vi "GT_Monitor.vi"() -> ()   [LabVIEW 2026]
doc: "Use this template to build a VI to use as a subVI."
panel:
  out "error out":errorcluster
  in  "stop":bool
  out "Right Step Text":string
  out "Status":T1
  in  "PLC Port":string
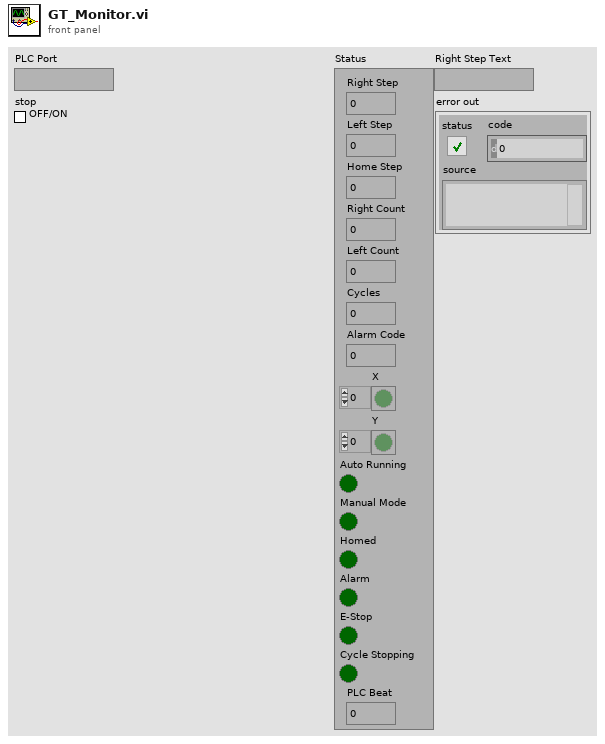
[diagram p1: front panel]
types:
  T1 = cluster{"Right Step":u16, "Left Step":u16, "Home Step":u16, "Right Count":u16, "Left Count":u16, "Cycles":u16, "Alarm Code":u16, "X":bool[], "Y":bool[], "Auto Running":bool, "Manual Mode":bool, "Homed":bool, "Alarm":bool, "E-Stop":bool, "Cycle Stopping":bool, "PLC Beat":u16}
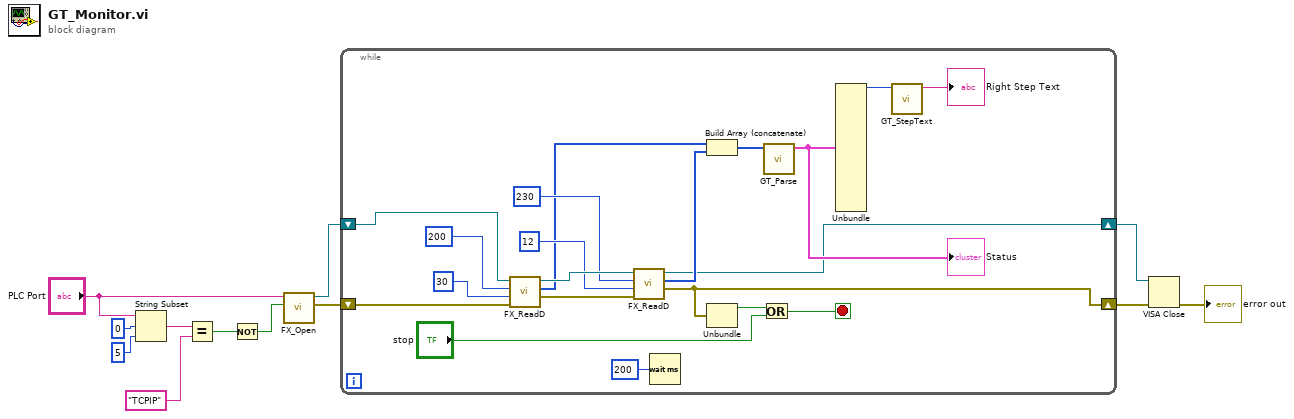
[diagram p0: block diagram]
diagram:
  n1 = String Subset(string="PLC Port", offset (0)=0, length (rest)=5 ("length (rest)")) -> (substring=w9:string)
  n2 = Equal?(x=w9, y="TCPIP") -> (x = y?=w7:bool)
  n3 = Not(x=w7) -> (.not. x?=w6:bool)
  n4 = call "FX_Open.vi"("Serial (COM)?"=w6, "Resource"="PLC Port") -> ("error out"=w4:errorcluster, "VISA out"=w5:refnum<visa-resource-name>)  [unwired: 8 in]
  n5 = while {
    shift-right: [w18] -> w3
    shift-left: w5 -> [w32]
    shift-right: [w17] -> w2
    shift-left: w4 -> [w31]
    stop <- w14 stop-if-true
    n6 = call "FX_ReadD.vi"("error in (no error)"=w31, "Count"=u16 30, "D"=u16 200, "VISA in"=w32) -> ("error out"=w27:errorcluster, "Words"=w24:u16[], "VISA out"=w28:refnum<visa-resource-name>)  [unwired: 5 in]
    n7 = call "FX_ReadD.vi"("error in (no error)"=w27, "Count"=u16 12, "D"=u16 230, "VISA in"=w28) -> ("error out"=w17:errorcluster, "Words"=w23:u16[], "VISA out"=w18:refnum<visa-resource-name>)  [unwired: 5 in]
    n8 = Wait (ms)(milliseconds to wait=u32 200) -> ()  [unwired: 1 out]
    n9 = Build Array (concatenate)(w24, w23) -> (w22:u16[])
    n10 = Unbundle(w17) -> ("status"=w16:bool)  [unwired: 2 out]
    n11 = Or(x=w16, y="stop") -> (x .or. y?=w14:bool)
    n12 = call "GT_Parse.vi"("Words"=w22) -> ("Status"=w21:T1)  [unwired: 10 in]
    "Status" <- w21
    n13 = Unbundle(w21) -> ("Right Step"=w20:u16)  [unwired: 15 out]
    n14 = call "GT_StepText.vi"("Step"=w20) -> ("Step Text"=→"Right Step Text":string)  [unwired: 10 in]
  }
  n15 = VISA Close(VISA resource name=w3, error in (no error)=w2) -> (error out=→"error out":errorcluster)
